vi "Event Handler.vi"(0 "uService Template in":refnum<class "Scheduler.lvclass">, 5 "Event type":T1=enum."Message", 7 "Item Name":string, 9 "Data":variant, 11 "error in (no error)":errorcluster) -> (4 "uService Template out":refnum<class "Scheduler.lvclass">, 15 "error out":errorcluster)   [LabVIEW 2020, in "Scheduler.lvlib" / "Scheduler.lvclass"]
doc: "This VI is the event handler of the uService: every time an event is triggered to the uService, this VI is called.\nNote: here you can access the Actor/Class data, but it will be the one coming out from Init. You cannot modify the values.\nThree different events are supported:\nI) Button Pressed: get called on a GUI button pressed. Item Name is the name (label) of the button, Data is empty.\nII) Shared Variable Updated: get called when a SV you subscribed to is updated. Item Name is the name of the SV, and Data is the value (note: you need to convert it to the proper type).\nIII) Message: get called every time a user event is generated using Send Message to Event Handler. The values of Item Name and Data are the one given to the Send Message to Event Handler.\nIV) Ready to launch?: this frame get called every time a new Run is initiated. Each uService is responsible of performing a self check before giving back the green light for the Run to start."
uses:
  Scheduler.lvclass
  TALOS/TALOS_PPL.lvlibp/Father of all uServices/Father of all uServices/Event Handler Items.ctl
  Scheduler Consumer Case Selector.ctl
  Append Options.ctl
  Run Utilities/Schedule/Schedule.lvclass
  Run Utilities/Sequence of SBlocks/Sequence of SBlocks.lvclass
  Add RUN Window.vi
  Preview.vi
  Get File Path for Load and Save.vi
  TALOS/TALOS_PPL.lvlibp/Father of all uServices/Father of all uServices/Father of all uServices.lvclass
  Scheduler.lvclass/Scheduler.ctl
  C:/LabVIEW Code/CIRCUS/TALOS/TALOS_PPL.lvlibp/Father of all uServices/Father of all uServices/Father of all uServices.lvclass
  TALOS/TALOS_PPL.lvlibp
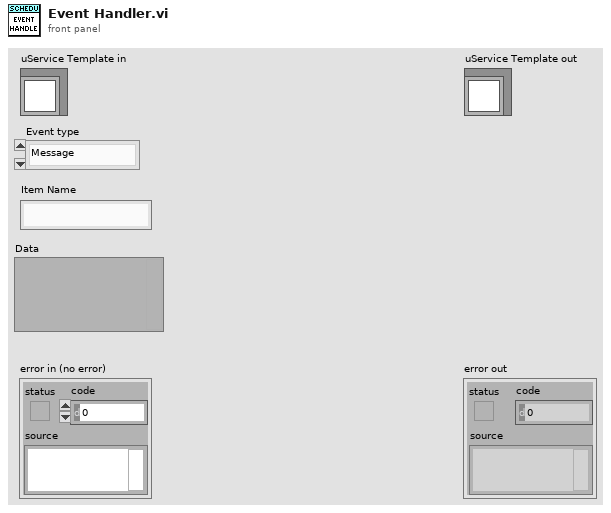
[diagram p1: front panel]
types:
  T1 = typedef "TALOS_PPL.lvlibp/Father of all uServices.lvlib/Father of all uServices.lvclass/Event Handler Items.ctl" = enum16{"Button Pressed", "Message", "Ready to launch?", "Safe Mode", "Start RUN", "Stop RUN"}
  T2 = enum32{"Invalid", "Standard", "Closed", "Hidden", "Minimized", "Maximized"}
  T3 = typedef "Scheduler.lvlib/Scheduler.lvclass/Scheduler Consumer Case Selector.ctl" = enum16{"Add SBlock", "Update GUI", "Move SBlock", "Select SBlock", "Update Cont.", "Load", "Save", "Reset", "Send to Tamer", "Edit SBlock", "Duplicate SBlock", "Delete SBlock", "Update SBlock", "Init", "Split/Combine Schedules", "Reschedule", "Load Parameters"}
  T4 = typedef "Scheduler.lvlib/Scheduler.lvclass/Append Options.ctl" = enum16{"New session", "Append to bottom", "Append to top"}
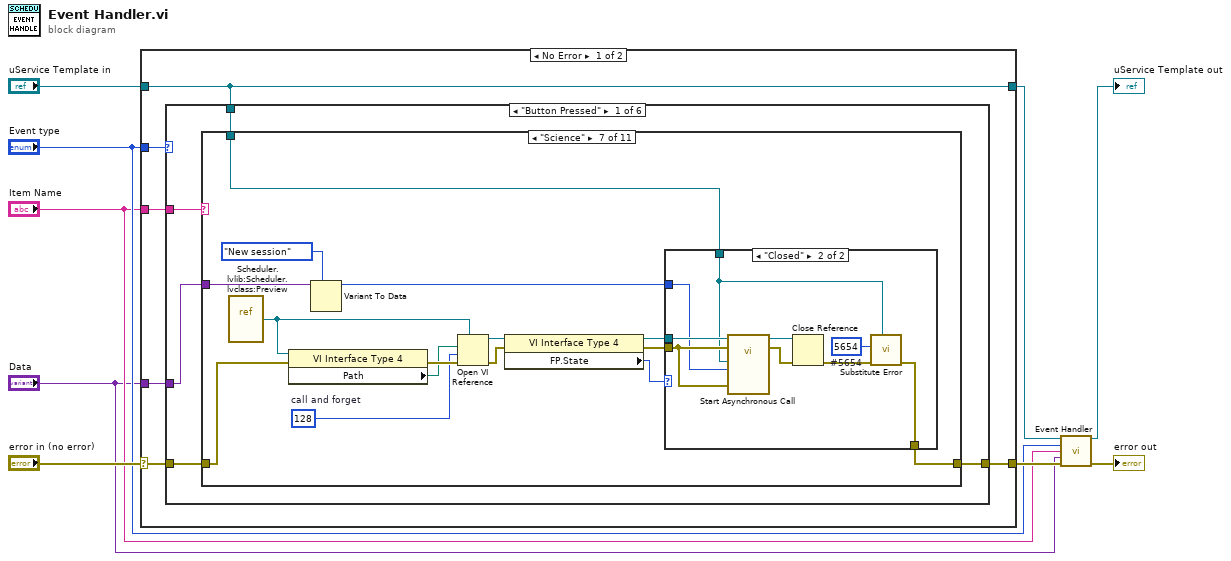
[diagram p0: block diagram]
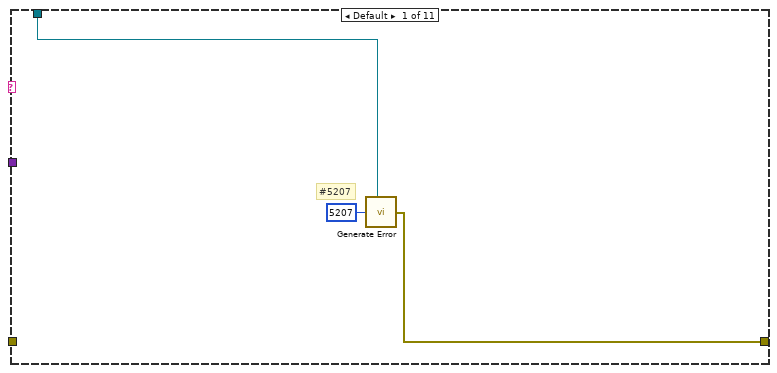
[diagram p2: hidden frame]
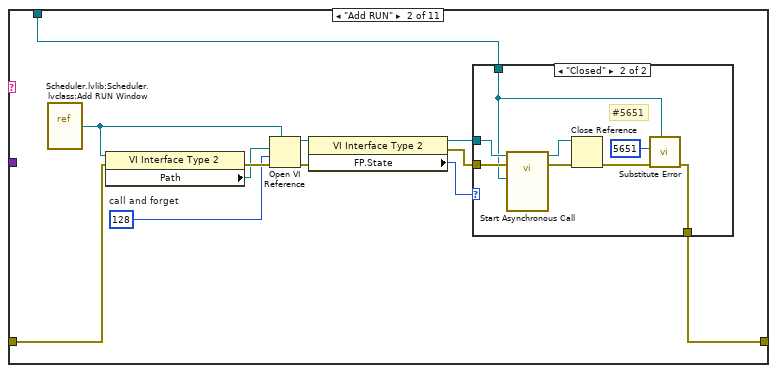
[diagram p3: hidden frame]
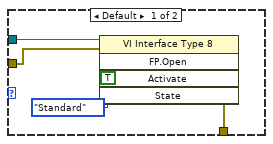
[diagram p4: hidden frame]
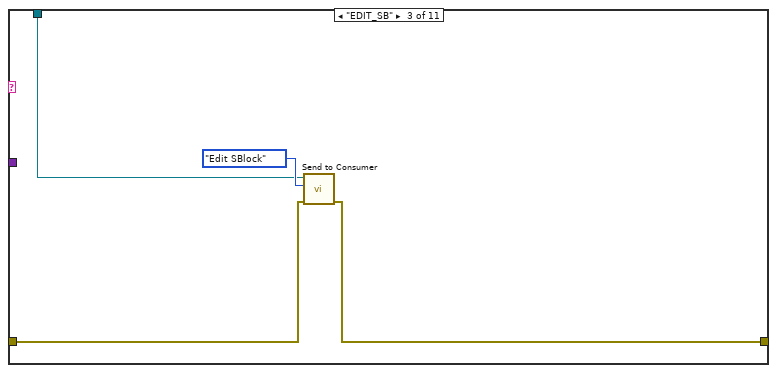
[diagram p5: hidden frame]
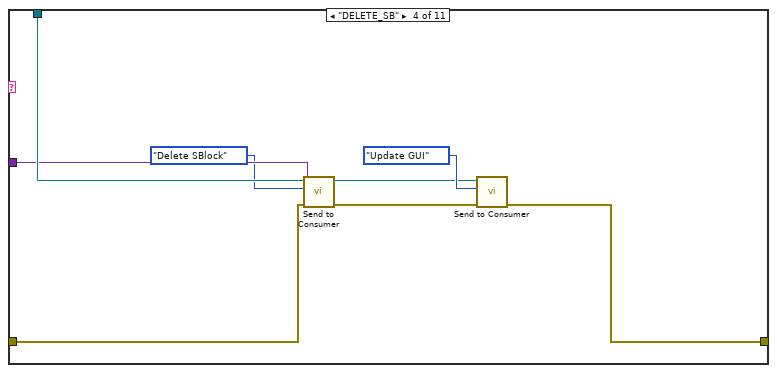
[diagram p6: hidden frame]
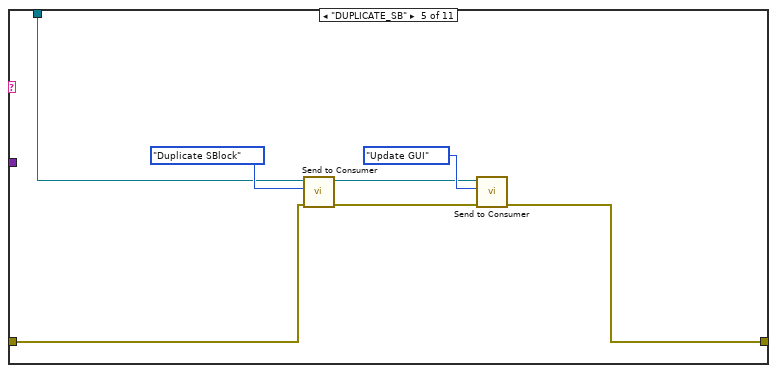
[diagram p7: hidden frame]
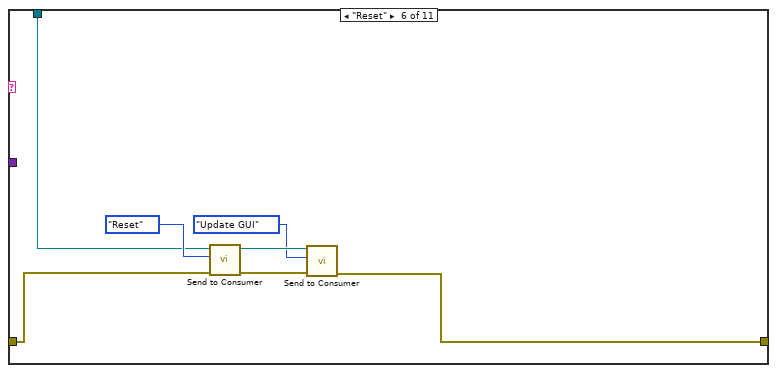
[diagram p8: hidden frame]
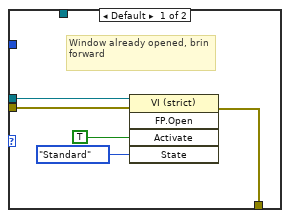
[diagram p9: hidden frame]
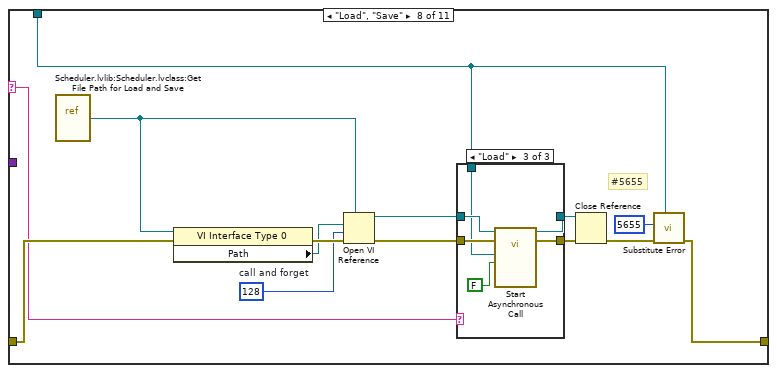
[diagram p10: hidden frame]
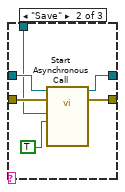
[diagram p12: hidden frame]
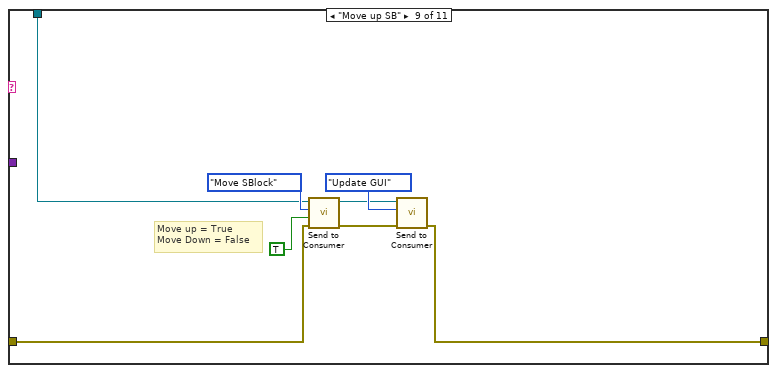
[diagram p13: hidden frame]
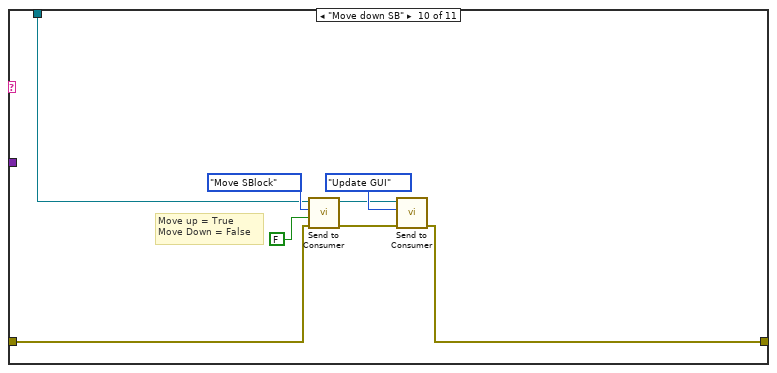
[diagram p14: hidden frame]
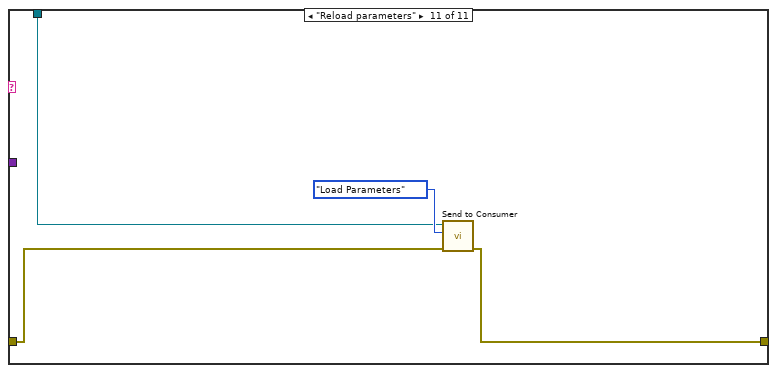
[diagram p15: hidden frame]
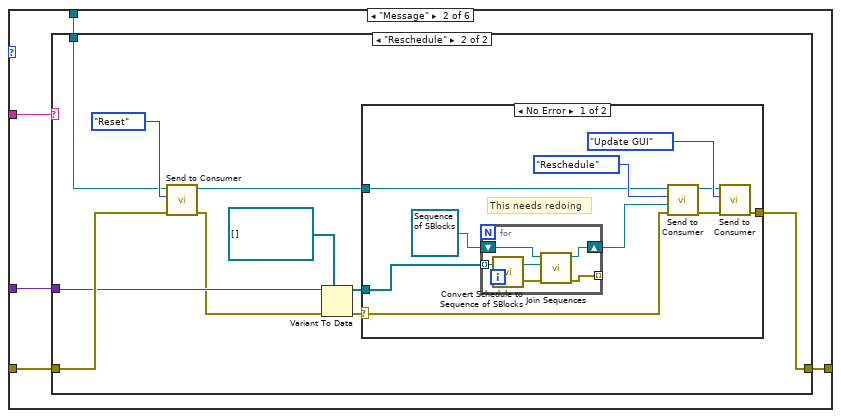
[diagram p16: hidden frame]
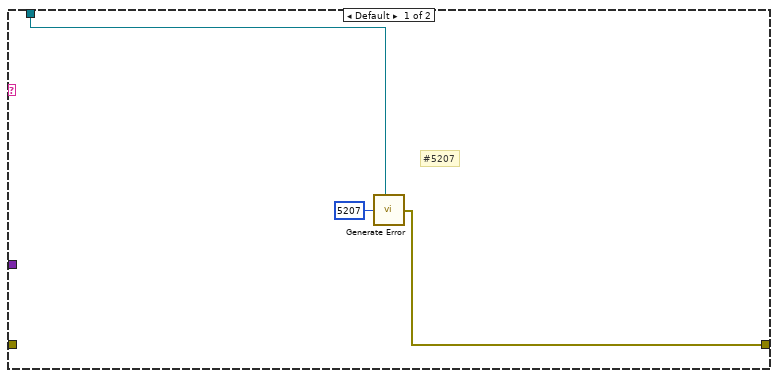
[diagram p17: hidden frame]
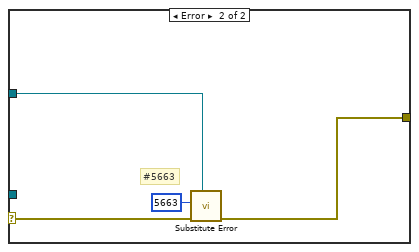
[diagram p18: hidden frame]
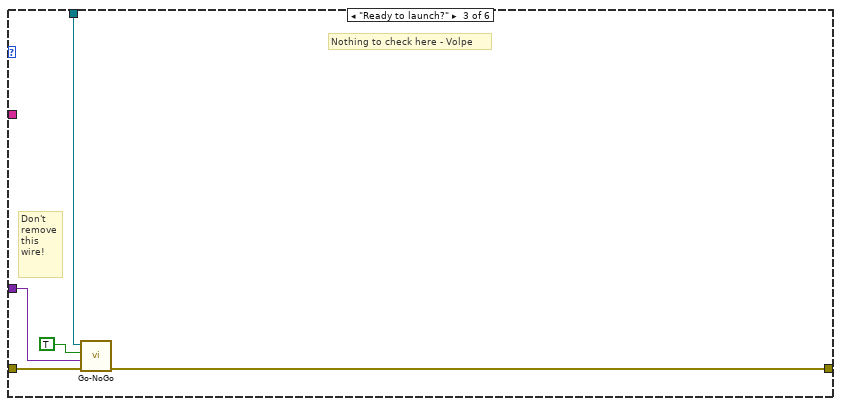
[diagram p19: hidden frame]
diagram:
  n1 = case shown="No Error" "error in (no error)" {
    selector: "error in (no error)" -> [w13 w199]
    tunnel: [w14 w199] -> w7
    tunnel: [w12 w198] -> w4
    tunnel: "uService Template in" -> [w12 w198]
    tunnel: "Event type" -> [w15 _]
    tunnel: "Item Name" -> [w11 _]
    tunnel: "Data" -> [w10 _]
    frame No Error {
      n2 = case shown="\"Button Pressed\"" w15 {
        tunnel: [w20 w152 w193 w195 w196 w197] -> w14
        tunnel: w13 -> [w17 w156 w194 w195 w196 w197]
        tunnel: w11 -> [w18 w155 _ _ _ _]
        tunnel: w12 -> [w19 w153 w192 _ _ _]
        tunnel: w10 -> [w16 w154 w190 _ _ _]
        frame "Button Pressed" {
          n3 = case shown="\"Science\"" w18 {
            selector: w18 -> [_ _ _ _ _ _ _ w105 _ _ _]
            tunnel: w17 -> [_ w28 w52 w60 w67 w73 w85 w109 w137 w145 w151]
            tunnel: [w21 w31 w51 w54 w63 w70 w82 w106 w136 w144 w150] -> w20
            tunnel: w19 -> [w22 w32 w49 w59 w62 w69 w84 w108 w134 w142 w148]
            tunnel: w16 -> [_ _ _ w58 _ _ w77 _ _ _ _]
            frame Default {
              # "#5207"
              n4 = call "Generate Error.vi"("Class"=w22, "Error Code"=5207) -> ("error out"=w21:errorcluster)  [unwired: 5 in]
            }
            frame "Add RUN" {
              w33 = 128  # call and forget
              n5 = vi-ref "Scheduler.lvlib:Scheduler.lvclass:Add RUN Window.vi"() -> (w30:refnum<vi>)
              n6 = property class="VI Interface Type 2"(reference=w30, error in=w28) -> (error out=w35:errorcluster, "Path"=w29:path)  [unwired: 1 out]
              n7 = Open VI Reference(type specifier VI Refnum (for type only)=w30, vi path=w29, options=w33, error in (no error)=w35) -> (vi reference=w34:refnum<vi>, error out=w26:errorcluster)  [unwired: 2 in]
              n8 = property class="VI Interface Type 2"(reference=w34, error in=w26) -> (reference out=w27:refnum<vi>, error out=w25:errorcluster, "FP.State"=w24:T2)
              n9 = case shown="\"Closed\"" w24 {
                tunnel: w25 -> [w39 w48]
                tunnel: w27 -> [w40 w46]
                tunnel: w32 -> [_ w41]
                tunnel: [w38 w43] -> w31
                frame Default {
                  n10 = invoke class="VI Interface Type 8" method="FP.Open"(reference=w40, error in=w39, "Activate"=TRUE ("Activate?"), "State"=T2."Standard") -> (error out=w38:errorcluster)  [unwired: 1 in, 4 out]
                }
                frame "Closed" {
                  # "#5651"
                  n11 = call-by-ref "Start Asynchronous Call"(reference=w46, error in=w48, "CIRCUS_uServices.lvlib:Scheduler.lvlib:Scheduler.lvclass"=w41) -> (reference out=w45:refnum<vi>, error out=w47:errorcluster)  [unwired: 9 in, 2 out]
                  n12 = Close Reference(reference=w45, error in (no error)=w47) -> (error out=w44:errorcluster)
                  n13 = call "Substitute Error.vi"("LabVIEW Object"=w41, "error in (no error)"=w44, "Error Code"=5651) -> ("error out"=w43:errorcluster)  [unwired: 8 in]
                }
              }
            }
            frame "EDIT_SB" {
              n14 = call "Send to Consumer.vi"("error in (no error)"=w52, "Case ID"=Scheduler_Consumer_Case_Selector."Edit SBlock" ("Shifter Panel Consumer Case Selector"), "uService Template in"=w49) -> ("error out"=w51:errorcluster)  [unwired: 7 in, 1 out]
            }
            frame "DELETE_SB" {
              n15 = call "Send to Consumer.vi"("error in (no error)"=w60, "Data"=w58, "Case ID"=Scheduler_Consumer_Case_Selector."Delete SBlock" ("Shifter Panel Consumer Case Selector"), "uService Template in"=w59) -> ("error out"=w55:errorcluster, "uService Template out"=w53:refnum<class "Scheduler.lvclass">)  [unwired: 6 in]
              n16 = call "Send to Consumer.vi"("error in (no error)"=w55, "Case ID"=Scheduler_Consumer_Case_Selector."Update GUI" ("Shifter Panel Consumer Case Selector"), "uService Template in"=w53) -> ("error out"=w54:errorcluster)  [unwired: 7 in, 1 out]
            }
            frame "DUPLICATE_SB" {
              n17 = call "Send to Consumer.vi"("error in (no error)"=w67, "Case ID"=Scheduler_Consumer_Case_Selector."Duplicate SBlock" ("Shifter Panel Consumer Case Selector"), "uService Template in"=w62) -> ("error out"=w64:errorcluster, "uService Template out"=w61:refnum<class "Scheduler.lvclass">)  [unwired: 7 in]
              n18 = call "Send to Consumer.vi"("error in (no error)"=w64, "Case ID"=Scheduler_Consumer_Case_Selector."Update GUI" ("Shifter Panel Consumer Case Selector"), "uService Template in"=w61) -> ("error out"=w63:errorcluster)  [unwired: 7 in, 1 out]
            }
            frame "Reset" {
              n19 = call "Send to Consumer.vi"("error in (no error)"=w73, "Case ID"=Scheduler_Consumer_Case_Selector."Reset" ("Shifter Panel Consumer Case Selector"), "uService Template in"=w69) -> ("error out"=w71:errorcluster, "uService Template out"=w72:refnum<class "Scheduler.lvclass">)  [unwired: 7 in]
              n20 = call "Send to Consumer.vi"("error in (no error)"=w71, "Case ID"=Scheduler_Consumer_Case_Selector."Update GUI" ("Shifter Panel Consumer Case Selector"), "uService Template in"=w72) -> ("error out"=w70:errorcluster)  [unwired: 7 in, 1 out]
            }
            frame "Science" {
              w86 = 128  # call and forget
              n21 = vi-ref "Scheduler.lvlib:Scheduler.lvclass:Preview.vi"() -> (w83:refnum<vi>)
              n22 = property class="VI Interface Type 4"(reference=w83, error in=w85) -> (error out=w89:errorcluster, "Path"=w88:path)  [unwired: 1 out]
              n23 = Variant To Data(type=Append_Options."New session" ("Append"), Variant=w77) -> (data=w75:T4)  [unwired: 1 in, 1 out]
              n24 = Open VI Reference(type specifier VI Refnum (for type only)=w83, vi path=w88, options=w86, error in (no error)=w89) -> (vi reference=w87:refnum<vi>, error out=w80:errorcluster)  [unwired: 2 in]
              n25 = property class="VI Interface Type 4"(reference=w87, error in=w80) -> (reference out=w81:refnum<vi>, error out=w79:errorcluster, "FP.State"=w78:T2)
              n26 = case shown="\"Closed\"" w78 {
                tunnel: w84 -> [_ w96]
                tunnel: [w90 w99] -> w82
                tunnel: w81 -> [w92 w97]
                tunnel: w79 -> [w91 w103]
                tunnel: w75 -> [_ w95]
                frame Default {
                  # "Window already opened, brin forward"
                  n27 = invoke class="VI (strict)" method="FP.Open"(reference=w92, error in=w91, "Activate"=TRUE ("Activate?"), "State"=T2."Standard") -> (error out=w90:errorcluster)  [unwired: 1 in, 4 out]
                }
                frame "Closed" {
                  w98 = 5654  # #5654
                  n28 = call-by-ref "Start Asynchronous Call"(reference=w97, error in=w103, 8:"error in (no error)"=w103, "Append"=w95, "Scheduler in"=w96) -> (reference out=w101:refnum<vi>, error out=w100:errorcluster)  [unwired: 7 in, 2 out]
                  n29 = Close Reference(reference=w101, error in (no error)=w100) -> (error out=w102:errorcluster)
                  n30 = call "Substitute Error.vi"("LabVIEW Object"=w96, "error in (no error)"=w102, "Error Code"=w98) -> ("error out"=w99:errorcluster)  [unwired: 8 in]
                }
              }
            }
            frame "Load", "Save" {
              w110 = 128  # call and forget
              # "#5655"
              n31 = vi-ref "Scheduler.lvlib:Scheduler.lvclass:Get File Path for Load and Save.vi"() -> (w107:refnum<vi>)
              n32 = property class="VI Interface Type 0"(reference=w107, error in=w109) -> (error out=w117:errorcluster, "Path"=w116:path)  [unwired: 1 out]
              n33 = Open VI Reference(type specifier VI Refnum (for type only)=w107, vi path=w116, options=w110, error in (no error)=w117) -> (vi reference=w113:refnum<vi>, error out=w111:errorcluster)  [unwired: 2 in]
              n34 = case shown="\"Load\"" w105 {
                tunnel: [w119 w120 w131] -> w114
                tunnel: w113 -> [w119 w125 w130]
                tunnel: [w118 w124 w129] -> w112
                tunnel: w111 -> [w118 w123 w128]
                tunnel: w108 -> [_ w122 w127]
                frame Default {
                }
                frame "Save" {
                  n35 = call-by-ref "Start Asynchronous Call"(reference=w125, error in=w123, "Save/Load"=TRUE, "Scheduler in"=w122) -> (reference out=w120:refnum<vi>, error out=w124:errorcluster)  [unwired: 8 in, 2 out]
                }
                frame "Load" {
                  n36 = call-by-ref "Start Asynchronous Call"(reference=w130, error in=w128, "Save/Load"=FALSE, "Scheduler in"=w127) -> (reference out=w131:refnum<vi>, error out=w129:errorcluster)  [unwired: 8 in, 2 out]
                }
              }
              n37 = Close Reference(reference=w114, error in (no error)=w112) -> (error out=w115:errorcluster)
              n38 = call "Substitute Error.vi"("LabVIEW Object"=w108, "error in (no error)"=w115, "Error Code"=5655) -> ("error out"=w106:errorcluster)  [unwired: 8 in]
            }
            frame "Move up SB" {
              # "Move up = True\nMove Down = False"
              n39 = call "Send to Consumer.vi"("error in (no error)"=w137, "Data"=TRUE, "Case ID"=Scheduler_Consumer_Case_Selector."Move SBlock" ("Shifter Panel Consumer Case Selector"), "uService Template in"=w134) -> ("error out"=w135:errorcluster, "uService Template out"=w133:refnum<class "Scheduler.lvclass">)  [unwired: 6 in]
              n40 = call "Send to Consumer.vi"("error in (no error)"=w135, "Case ID"=Scheduler_Consumer_Case_Selector."Update GUI" ("Shifter Panel Consumer Case Selector"), "uService Template in"=w133) -> ("error out"=w136:errorcluster)  [unwired: 7 in, 1 out]
            }
            frame "Move down SB" {
              # "Move up = True\nMove Down = False"
              n41 = call "Send to Consumer.vi"("error in (no error)"=w145, "Data"=FALSE, "Case ID"=Scheduler_Consumer_Case_Selector."Move SBlock" ("Shifter Panel Consumer Case Selector"), "uService Template in"=w142) -> ("error out"=w143:errorcluster, "uService Template out"=w141:refnum<class "Scheduler.lvclass">)  [unwired: 6 in]
              n42 = call "Send to Consumer.vi"("error in (no error)"=w143, "Case ID"=Scheduler_Consumer_Case_Selector."Update GUI" ("Shifter Panel Consumer Case Selector"), "uService Template in"=w141) -> ("error out"=w144:errorcluster)  [unwired: 7 in, 1 out]
            }
            frame "Reload parameters" {
              n43 = call "Send to Consumer.vi"("error in (no error)"=w151, "Case ID"=Scheduler_Consumer_Case_Selector."Load Parameters" ("Shifter Panel Consumer Case Selector"), "uService Template in"=w148) -> ("error out"=w150:errorcluster)  [unwired: 7 in, 1 out]
            }
          }
        }
        frame "Message" {
          n44 = case shown="\"Reschedule\"" w155 {
            tunnel: w156 -> [_ w168]
            tunnel: w154 -> [_ w167]
            tunnel: w153 -> [w158 w160]
            tunnel: [w157 w169] -> w152
            frame Default {
              # "#5207"
              n45 = call "Generate Error.vi"("Class"=w158, "Error Code"=5207) -> ("error out"=w157:errorcluster)  [unwired: 5 in]
            }
            frame "Reschedule" {
              n46 = call "Send to Consumer.vi"("error in (no error)"=w168, "Case ID"=Scheduler_Consumer_Case_Selector."Reset" ("Shifter Panel Consumer Case Selector"), "uService Template in"=w160) -> ("error out"=w164:errorcluster, "uService Template out"=w166:refnum<class "Scheduler.lvclass">)  [unwired: 7 in]
              n47 = Variant To Data(error in=w164, type=refnum<class "Schedule.lvclass">[] [], Variant=w167) -> (data=w162:refnum<class "Schedule.lvclass">[], error out=w161:errorcluster)
              n48 = case shown="No Error" w161 {
                selector: w161 -> [w174 w187]
                tunnel: [w172 w188] -> w169
                tunnel: w166 -> [w178 w189]
                tunnel: w162 -> [w177 _]
                frame No Error {
                  # "This needs redoing"
                  n49 = for {
                    tunnel: w177 -> [w185] mode=indexing
                    shift-right: [w182] -> w175
                    shift-left: refnum<class "Sequence of SBlocks.lvclass"> refnum ("Sequence of SBlocks in") -> [w183]
                    tunnel: [w180] -> _ mode=indexing
                    n50 = call "Convert Schedule to Sequence of SBlocks.vi"("Schedule"=w185) -> ("error out"=w181:errorcluster, "Sequence of SBlocks"=w184:refnum<class "Sequence of SBlocks.lvclass">)  [unwired: 1 in]
                    n51 = call-dynamic "Join Sequences.vi"("error in (no error)"=w181, "Sequence of SBlocks"=w184, "Sequence of SBlocks in"=w183) -> ("error out"=w180:errorcluster, "Sequence of SBlocks out"=w182:refnum<class "Sequence of SBlocks.lvclass">)  [unwired: 7 in]
                  }
                  n52 = call "Send to Consumer.vi"("error in (no error)"=w174, "Data"=w175, "Case ID"=Scheduler_Consumer_Case_Selector."Reschedule" ("Shifter Panel Consumer Case Selector"), "uService Template in"=w178) -> ("error out"=w173:errorcluster, "uService Template out"=w170:refnum<class "Scheduler.lvclass">)  [unwired: 6 in]
                  n53 = call "Send to Consumer.vi"("error in (no error)"=w173, "Case ID"=Scheduler_Consumer_Case_Selector."Update GUI" ("Shifter Panel Consumer Case Selector"), "uService Template in"=w170) -> ("error out"=w172:errorcluster)  [unwired: 7 in, 1 out]
                }
                frame Error {
                  # "#5663"
                  n54 = call "Substitute Error.vi"("LabVIEW Object"=w189, "error in (no error)"=w187, "Error Code"=5663) -> ("error out"=w188:errorcluster)  [unwired: 8 in]
                }
              }
            }
          }
        }
        frame "Ready to launch?" {
          # "Nothing to check here - Volpe"
          # "Don't remove this wire!"
          n55 = call-dynamic "Go-NoGo.vi"("error in (no error)"=w194, "Go-NoGo Data"=w190, "Go?"=TRUE, "Father of all uServices in"=w192) -> ("error out"=w193:errorcluster)  [unwired: 6 in, 1 out]
        }
        frame "Safe Mode" {
          # "Do nothing - Volpe"
        }
        frame "Start RUN" {
        }
        frame "Stop RUN" {
        }
      }
    }
    frame Error {
    }
  }
  n56 = call-parent "Event Handler.vi"("uService Template in"=w4, "Event type"="Event type", "Item Name"="Item Name", "Data"="Data", "error in (no error)"=w7) -> ("uService Template out"=→"uService Template out":refnum<class "Scheduler.lvclass">, "error out"=→"error out":errorcluster)  [unwired: 9 in]
